vi "Get Case Structure Frame Index (by Name).vi"(8 "error in (no error)":errorcluster, 10 "element":string, 11 "CaseStructure in":refnum<vi>) -> (0 "error out":errorcluster, 1 "Found?":bool, 2 "Frame Index":i32, 3 "CaseStructure out":refnum<vi>)   [LabVIEW 2019, in "gRPC Template Creation Utility.lvlib"]
uses:
  gRPC Template Creation Utility.lvlib
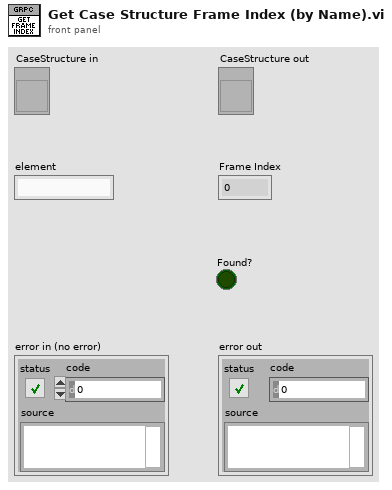
[diagram p1: front panel]
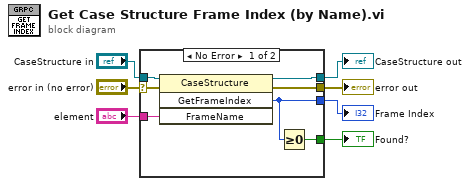
[diagram p0: block diagram]
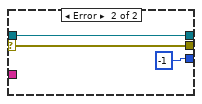
[diagram p2: hidden frame]
diagram:
  n1 = case shown="No Error" "error in (no error)" {
    selector: "error in (no error)" -> [w10 w17]
    tunnel: "CaseStructure in" -> [w14 w16]
    tunnel: [w13 w16] -> w6
    tunnel: [w11 w17] -> w5
    tunnel: "element" -> [w12 _]
    tunnel: [w9 _] -> w2
    tunnel: [w8 -1 ("GetFrameIndex")] -> w1
    frame No Error {
      n2 = invoke class="CaseStructure" method="GetFrameIndex"(reference=w14, error in=w10, "FrameName"=w12) -> (reference out=w13:refnum<vi>, error out=w11:errorcluster, "GetFrameIndex"=w8:i32)  [unwired: 1 in, 1 out]
      n3 = Greater Or Equal To 0?(x=w8) -> (x >= 0?=w9:bool)
    }
    frame Error {
    }
  }
  "CaseStructure out" <- w6
  "error out" <- w5
  "Found?" <- w2
  "Frame Index" <- w1
